vi "Gold--constant.vi"() -> (1 "Gold":u32(colorbox))   [LabVIEW 2018, in "Band Colors.lvlib"]
doc: "Provides the RGB color value for gold.\n\nThe VI converts the RGB components (212, 175, 55) into a LabVIEW color value and returns it through <b>Gold</b>."
uses:
  Band Colors.lvlib
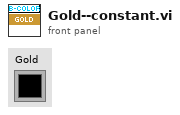
[diagram p1: front panel]
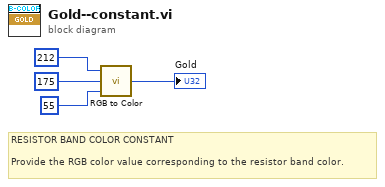
[diagram p0: block diagram]
diagram:
  # "RESISTOR BAND COLOR CONSTANT\n\nProvide the RGB color value corresponding to the resistor band color."
  n1 = call <vilib>:"RGB to Color.vi"("B"=u8 55, "G"=u8 175, "R"=u8 212) -> ("Color"=→"Gold":u32)
